vi "Window-Position control window.vi"() -> ()   [LabVIEW 2020]
uses:
  <userlib>/My Palettes.lib/Custom Controls/Directional Arrow Buttons/Arrow button-East.ctl
  <userlib>/My Palettes.lib/Custom Controls/Directional Arrow Buttons/Arrow button-West.ctl
  <userlib>/My Palettes.lib/Custom Controls/Directional Arrow Buttons/Arrow button-North.ctl
  <userlib>/My Palettes.lib/Custom Controls/Directional Arrow Buttons/Arrow button-South.ctl
  <userlib>/My Palettes.lib/Custom Controls/Directional Arrow Buttons/Arrow button-North west.ctl
  <userlib>/My Palettes.lib/Custom Controls/Directional Arrow Buttons/Arrow button-North east.ctl
  <userlib>/My Palettes.lib/Custom Controls/Directional Arrow Buttons/Arrow button-South west.ctl
  <userlib>/My Palettes.lib/Custom Controls/Directional Arrow Buttons/Arrow button-South east.ctl
  User Interface/Windows/Position control window/Typedefs/Pos Ctrl States.ctl
  User Interface/Windows/Position control window/Typedefs/Pos Ctrl queue data cluster.ctl
  User Interface/Windows/Position control window/Typedefs/Pos Ctrl window refs cluster.ctl
  Typedefs/Movement mode.ctl
  Peripherals Control/XYZ Stage/Typedefs/XYZ stage states.ctl
  Typedefs/Axis of movement.ctl
  User Interface/Windows/Position control window/Globals/Pos ctrl window globals.vi
  Global Variables/General Globals.vi
  Peripherals Control/XYZ Stage/Globals/gl_XYZStage globals.vi
  Typedefs/Save-Load enum.ctl
  Peripherals Control/XYZ Stage/Typedefs/XYZ channel ring.ctl
  Peripherals Control/XYZ Stage/Typedefs/XYZ stage data.ctl
panel:
  in  "Speed setting\navailable":bool
  in  "Motor E-Stop":bool
  out "# elements in queue":i32
  out "x+1":dbl
  in  "Y Coordinate ctrl":sgl min=-20000 max=20000 step=0.1 format="Y:%#_g um"
  out "Close":bool
  in  "Z step (um)":sgl=1.0 min=0.1 max=1000 step=0.1 format="%#_6f"
  in  "Z Coordinate ctrl":sgl min=-20000 max=20000 step=0.1 format="Z:%#.1f um"
  in  "Z move down":T1
  in  "Z move up":T2
  out "Z-axis section":string
  in  "Step = size of image":bool
  in  "XY step (um)":sgl=1.0 min=0.1 max=10000 step=0.1
  out "State":T3
  out "Last button name":string
  out "Event loop":i32
  out "Elapsed Time (s)":dbl format="%#.1g"
  in  "Speed setting ctrl":i32=1000 min=1000 max=50000 step=1 format="Speed\n%#_6g\num/sec"
  in  "Speed down":bool
  in  "Speed up":bool
  in  "X Coordinate ctrl":sgl min=-20000 max=20000 step=0.1 format="X:%#_g um"
  in  "Down-right":T4
  in  "Down-left":T5
  in  "Up-right":T6
  in  "Up-left":T7
  in  "Down":T1
  in  "Up":T2
  in  "Left":T8
  in  "Right":T9
  # "Speed"
  # "X-Y Movement"
  # "Z Movement"
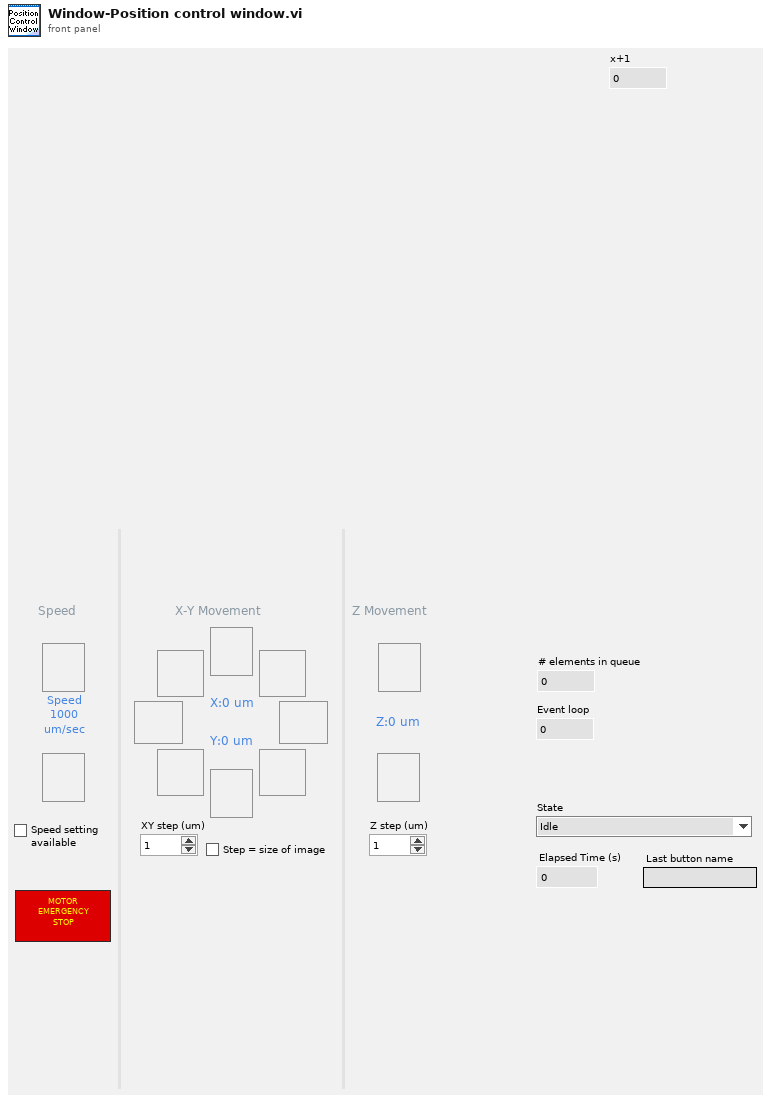
[diagram p1: front panel]
types:
  T1 = typedef "Arrow button-South.ctl" = bool
  T2 = typedef "Arrow button-North.ctl" = bool
  T3 = typedef "Pos Ctrl States.ctl" = enum16{"Idle", "Count-down", "Request single step (ack.)", "Request single step (no ack.)", "Request continuous movement", "Request movement stop"}
  T4 = typedef "Arrow button-South east.ctl" = bool
  T5 = typedef "Arrow button-South west.ctl" = bool
  T6 = typedef "Arrow button-North east.ctl" = bool
  T7 = typedef "Arrow button-North west.ctl" = bool
  T8 = typedef "Arrow button-West.ctl" = bool
  T9 = typedef "Arrow button-East.ctl" = bool
  T10 = typedef "Pos Ctrl window refs cluster.ctl" = cluster{"menu reference":refnum<k9>, "X Coordinate ctrl":refnum<vi>, "Y Coordinate ctrl":refnum<vi>, "Z Coordinate ctrl":refnum<vi>, "Speed setting ctrl":refnum<vi>, "Up":refnum<vi>, "Down":refnum<vi>, "Left":refnum<vi>, "Right":refnum<vi>, "Z move up":refnum<vi>, "Z move down":refnum<vi>, "Down-left":refnum<vi>, "Down-right":refnum<vi>, "Up-left":refnum<vi>, "Up-right":refnum<vi>, "Step = size of image":refnum<vi>, "XY step (um)":refnum<vi>, "Z step (um)":refnum<vi>, "Speed setting\navailable":refnum<vi>}
  T11 = typedef "Pos Ctrl queue data cluster.ctl" = cluster{"State":T3, "variant":variant}
  T12 = enum32{"Invalid", "Standard", "Closed", "Hidden", "Minimized", "Maximized"}
  T13 = typedef "XYZ stage states.ctl" = enum16{"Dequeue", "Initialize", "Read Position", "Read Speed Setting", "Move", "Set Max Speed", "Reset Axis", "Stop all movement"}
  T14 = typedef "Axis of movement.ctl" = enum16{"None", "X-axis", "Y-Axis", "-45 deg Axis", "+45 deg Axis", "Z-Axis"}
  T15 = enum8{"Enabled", "Disabled", "Disabled and Grayed Out"}
  T16 = typedef "XYZ stage data.ctl" = cluster{"Command":T13, "Channel":T17, "X":sgl, "Y":sgl, "Z":sgl, "Speed":i32, "Zero":bool, "Use acknowledgement?":bool}
  T17 = typedef "XYZ channel ring.ctl" = string
  T18 = typedef "Save-Load enum.ctl" = enum16{"Save to file", "Load from file", "Compare from file", "Save Backup"}
  T19 = typedef "Movement mode.ctl" = enum16{"Move the frame", "Move the feature"}
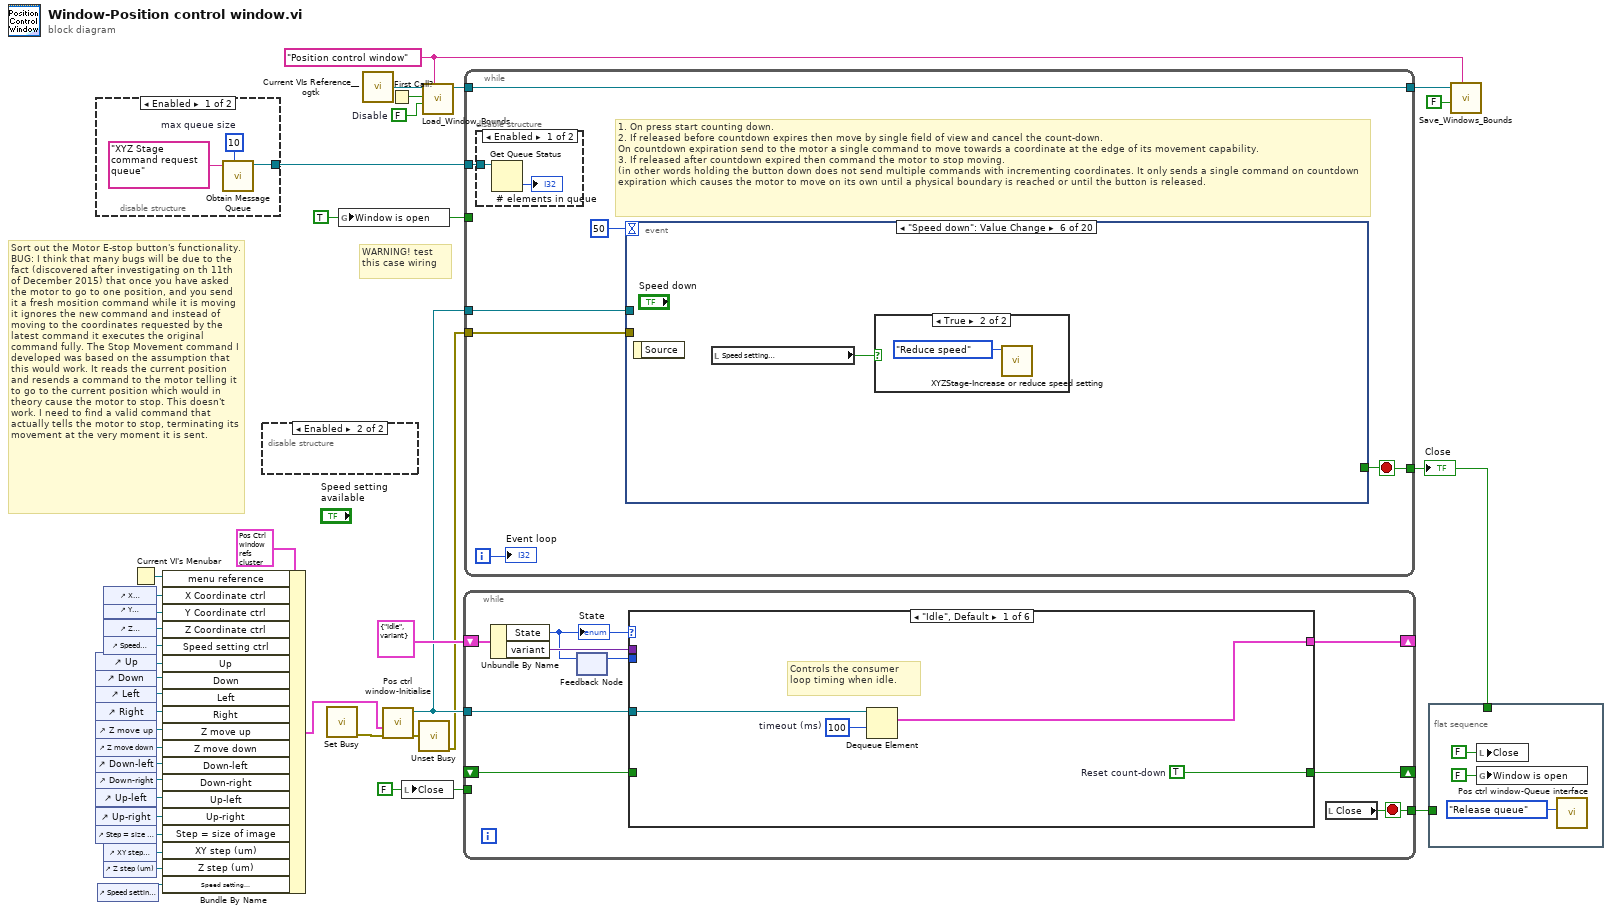
[diagram p0: block diagram]
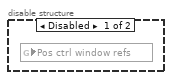
[diagram p3: hidden frame]
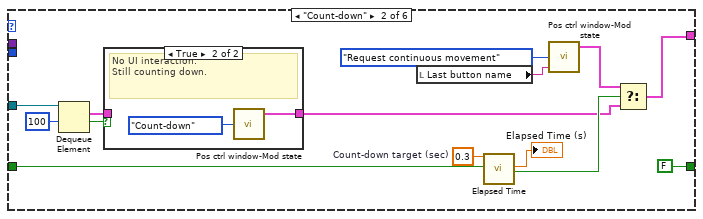
[diagram p4: hidden frame]
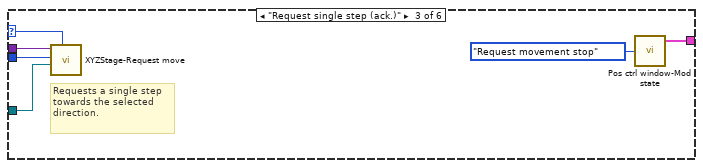
[diagram p6: hidden frame]
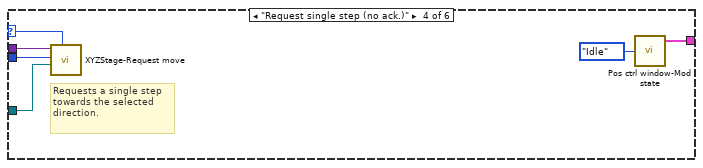
[diagram p7: hidden frame]
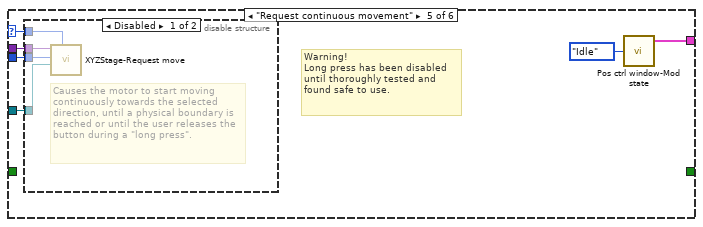
[diagram p8: hidden frame]
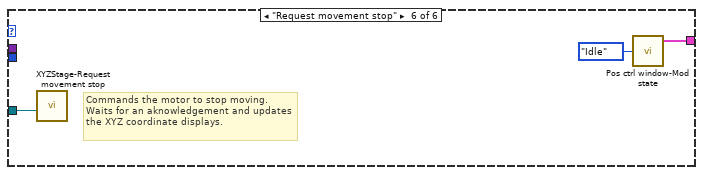
[diagram p10: hidden frame]
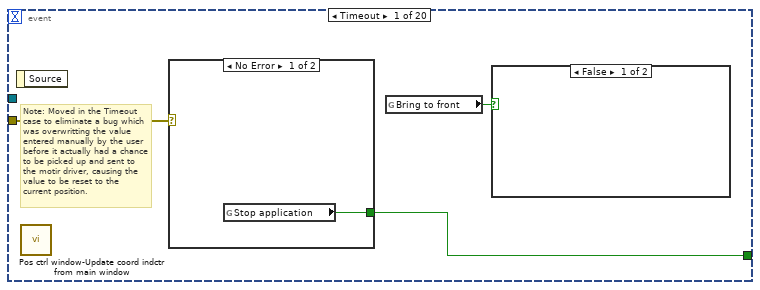
[diagram p12: hidden frame]
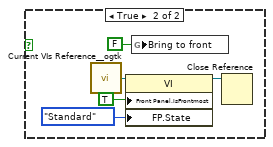
[diagram p13: hidden frame]
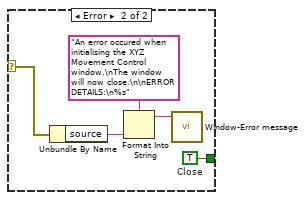
[diagram p14: hidden frame]
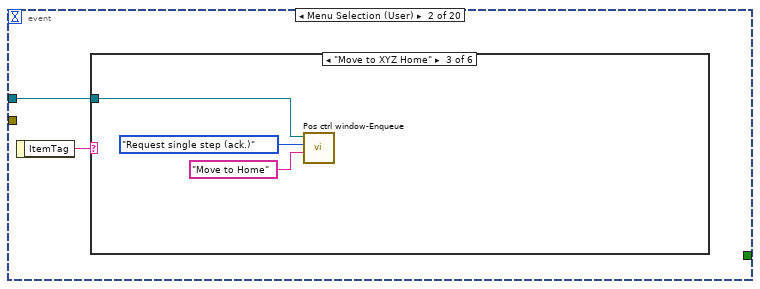
[diagram p15: hidden frame]
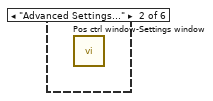
[diagram p17: hidden frame]
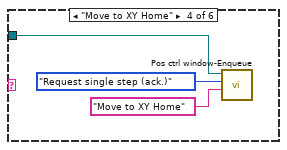
[diagram p18: hidden frame]
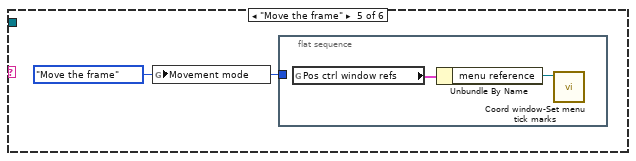
[diagram p19: hidden frame]
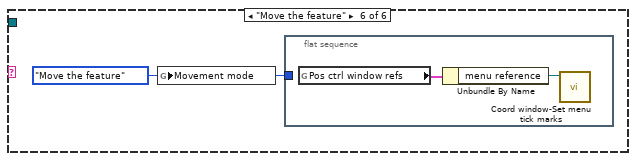
[diagram p20: hidden frame]
diagram:
  w11 = FALSE  # Disable
  w9 = "Position control window" ("Window Name (i.e. Key)")
  w15 = TRUE ("Bring to front")
  w26 = FALSE ("Close")
  # "Sort out the Motor E-stop button's functionality.\nBUG: I think that many bugs will be due to the fact (discovered after investigating on th 11th of December 2015) that once you have asked the motor to go to one position, and you send it a fresh mosition command while it is moving it ignores the new command and instead of moving to the coordinates requested by the latest command it executes the original command fully. The Stop Movement command I developed was based on the assumption that this would work. It reads the current position and resends a command to the motor telling it to go to the current position which would in theory cause the motor to stop. This doesn't work. I need to find a valid command that actually tells the motor to stop, terminating its movement at the very moment it is sent."
  # "WARNING! test this case wiring"
  n1 = control-ref of="Up"() -> (w36:refnum<vi>)
  n2 = control-ref of="Down"() -> (w35:refnum<vi>)
  n3 = control-ref of="Left"() -> (w34:refnum<vi>)
  n4 = control-ref of="Right"() -> (w33:refnum<vi>)
  n5 = control-ref of="Z move up"() -> (w32:refnum<vi>)
  n6 = control-ref of="Z move down"() -> (w31:refnum<vi>)
  n7 = control-ref of="Down-left"() -> (w30:refnum<vi>)
  n8 = control-ref of="Down-right"() -> (w29:refnum<vi>)
  n9 = control-ref of="Up-left"() -> (w28:refnum<vi>)
  n10 = control-ref of="Up-right"() -> (w27:refnum<vi>)
  n11 = control-ref of="Step = size of image"() -> (w24:refnum<vi>)
  n12 = disable-structure shown="Enabled" {
    disable-tunnel: [w39 _] -> w7
    frame Enabled {
      w41 = 10  # max queue size
      n13 = call "Obtain Message Queue.vi"("max queue size (-1, unlimited)"=w41, "Queue name"="XYZ Stage command request queue") -> ("Message Queue"=w39:refnum<queue>)  [unwired: 8 in, 1 out]
    }
    frame Disabled {
    }
  }
  n14 = control-ref of="Speed setting\navailable"() -> (w1:refnum<vi>)
  n15 = control-ref of="X Coordinate ctrl"() -> (w19:refnum<vi>)
  n16 = control-ref of="Y Coordinate ctrl"() -> (w18:refnum<vi>)
  n17 = control-ref of="Z Coordinate ctrl"() -> (w17:refnum<vi>)
  n18 = control-ref of="Speed setting ctrl"() -> (w16:refnum<vi>)
  n19 = control-ref of="XY step (um)"() -> (w23:refnum<vi>)
  n20 = control-ref of="Z step (um)"() -> (w22:refnum<vi>)
  n21 = Current VI's Menubar() -> (w6:refnum<k9>)
  n22 = Bundle By Name(cluster=T10 {"menu reference"=refnum, "X Coordinate ctrl"=refnum, "Y Coordinate ctrl"=refnum, "Z Coordinate ctrl"=refnum, "Speed setting ctrl"=refnum, "Up"=refnum, "Down"=refnum, "Left"=refnum, "Right"=refnum, "Z move up"=refnum, "Z move down"=refnum, "Down-left"=refnum, "Down-right"=refnum, "Up-left"=refnum, "Up-right"=refnum, "Step = size of image"=refnum, "XY step (um)"=refnum, "Z step (um)"=refnum, "Speed setting\navailable"=refnum} ("Pos ctrl window refs"), "menu reference"=w6, "X Coordinate ctrl"=w19, "Y Coordinate ctrl"=w18, "Z Coordinate ctrl"=w17, "Speed setting ctrl"=w16, "Up"=w36, "Down"=w35, "Left"=w34, "Right"=w33, "Z move up"=w32, "Z move down"=w31, "Down-left"=w30, "Down-right"=w29, "Up-left"=w28, "Up-right"=w27, "Step = size of image"=w24, "XY step (um)"=w23, "Z step (um)"=w22, "Speed setting\navailable"=w1) -> (w20:T10)
  n23 = disable-structure shown="Enabled" {
    frame Disabled {
      n24 = global read "Pos ctrl window globals.vi" "Pos ctrl window refs"() -> ()  [unwired: 1 in]
    }
    frame Enabled {
    }
  }
  n25 = call <vilib>:"Set Busy.vi"() -> ("error out"=w4:errorcluster)  [unwired: 10 in, 1 out]
  n26 = global write "Pos ctrl window globals.vi" "Window is open"(w15) -> ()
  n27 = call <userlib>:"Current VIs Reference__ogtk.vi"() -> ("Current VI's reference"=w14:refnum<vi>)  [unwired: 5 in]
  n28 = call "Pos ctrl window-Initialise.vi"("error in (no error)"=w4, "Pos ctrl window refs"=w20) -> ("error out"=w3:errorcluster, "XYZ movement ctrl window queue ref"=w21:refnum<queue>)  [unwired: 8 in]
  n29 = First Call?() -> (First Call?: T/F=w12:bool)
  n30 = local write "Close"(w26) -> ()
  n31 = call <vilib>:"Unset Busy.vi"("error in (no error)"=w3) -> ("error out"=w2:errorcluster)  [unwired: 10 in]
  n32 = call "Load_Window_Bounds.vi"("Window Name (i.e. Key)"=w9, "Disable"=w11, "First Call"=w12, "Window VI's Ref"=w14) -> ("reference out"=w13:refnum<vi>)  [unwired: 4 in, 3 out]
  n33 = while {
    tunnel: w21 -> [w50]
    shift-right: [w49] -> _
    shift-left: T11 {"State"=enum."Idle", "variant"=variant} ("Pos Ctrl queue data cluster") -> [w46]
    shift-right: [w48] -> _
    shift-left: _ -> [w47]
    tunnel: w26 -> [_]
    tunnel: [w42] -> w25
    stop <- w42 stop-if-true
    n34 = Unbundle By Name(w46) -> ("State"=w44:T3, "variant"=w45:variant)
    "State" <- w44
    n35 = feedback-in #1(w44) -> ()
    n36 = feedback #1() -> (w43:T3)  [unwired: 1 in]
    n37 = case shown="\"Idle\", Default" w44 {
      selector: w44 -> [_ _ w72 w78 w84 _]
      tunnel: w50 -> [w53 w67 w74 w80 w87 w94]
      tunnel: [w51 w56 w76 w82 w88 w95] -> w49
      tunnel: [w52 FALSE _ _ _ _] -> w48
      tunnel: w47 -> [_ w64 _ _ _ _]
      tunnel: w45 -> [_ _ w75 w81 w86 _]
      tunnel: w43 -> [_ _ w73 w79 w85 _]
      frame "Idle", Default {
        w52 = TRUE  # Reset count-down
        w54 = 100  # timeout (ms)
        # "Controls the consumer loop timing when idle."
        n38 = Dequeue Element(queue=w53, timeout in ms (-1)=w54) -> (element=w51:T11)  [unwired: 1 in, 3 out]
      }
      frame "Count-down" {
        w65 = 0.3  # Count-down target (sec)
        n39 = Dequeue Element(queue=w67, timeout in ms (-1)=100) -> (element=w62:T11, timed out?=w63:bool)  [unwired: 1 in, 2 out]
        n40 = case shown="True" w63 {
          tunnel: [w69 w70] -> w57
          tunnel: w62 -> [w69 _]
          frame False {
            # "Queue element received.\nUI interaction detected."
          }
          frame True {
            # "No UI interaction.\nStill counting down."
            n41 = call "Pos ctrl window-Mod state.vi"("States"=Pos_Ctrl_States."Count-down") -> ("Modified queue element"=w70:T11)  [unwired: 4 in]
          }
        }
        n42 = local read "Last button name"() -> (w55:string)
        n43 = call "Elapsed Time"("Time Target (s)"=w65, "Reset"=w64) -> ("Elapsed Time (s)"=→"Elapsed Time (s)":dbl, "Time has Elapsed"=w58:bool)  [unwired: 10 in, 6 out]
        n44 = call "Pos ctrl window-Mod state.vi"("variant"=w55, "States"=Pos_Ctrl_States."Request continuous movement") -> ("Modified queue element"=w60:T11)  [unwired: 3 in]
        n45 = Select(t=w60, s=w58, f=w57) -> (s? t:f=w56:T11)
      }
      frame "Request single step (ack.)" {
        # "Requests a single step towards the selected direction."
        n46 = call "XYZStage-Request move.vi"("Current State"=w72, "Pos ctrl window queue"=w74, "Previous State"=w73, "variant"=w75) -> ()  [unwired: 8 in]
        n47 = call "Pos ctrl window-Mod state.vi"("States"=Pos_Ctrl_States."Request movement stop") -> ("Modified queue element"=w76:T11)  [unwired: 4 in]
      }
      frame "Request single step (no ack.)" {
        # "Requests a single step towards the selected direction."
        n48 = call "XYZStage-Request move.vi"("Current State"=w78, "Pos ctrl window queue"=w80, "Previous State"=w79, "variant"=w81) -> ()  [unwired: 8 in]
        n49 = call "Pos ctrl window-Mod state.vi"("States"=Pos_Ctrl_States."Idle") -> ("Modified queue element"=w82:T11)  [unwired: 4 in]
      }
      frame "Request continuous movement" {
        # "Warning!\nLong press has been disabled until thoroughly tested and found safe to use."
        n50 = disable-structure shown="Disabled" {
          disable-tunnel: w87 -> [w93 _]
          disable-tunnel: w86 -> [w92 _]
          disable-tunnel: w85 -> [w91 _]
          disable-tunnel: w84 -> [w90 _]
          frame Disabled {
            # "Causes the motor to start moving continuously towards the selected direction, until a physical boundary is reached or until the user releases the button during a \"long press\"."
            n51 = call "XYZStage-Request move.vi"("Current State"=w90, "Pos ctrl window queue"=w93, "Previous State"=w91, "variant"=w92) -> ()  [unwired: 8 in]
          }
          frame Enabled {
          }
        }
        n52 = call "Pos ctrl window-Mod state.vi"("States"=Pos_Ctrl_States."Idle") -> ("Modified queue element"=w88:T11)  [unwired: 4 in]
      }
      frame "Request movement stop" {
        # "Commands the motor to stop moving.\nWaits for an aknowledgement and updates the XYZ coordinate displays."
        n53 = call "XYZStage-Request movement stop.vi"("Pos ctrl window queue"=w94) -> ()  [unwired: 11 in]
        n54 = call "Pos ctrl window-Mod state.vi"("States"=Pos_Ctrl_States."Idle") -> ("Modified queue element"=w95:T11)  [unwired: 4 in]
      }
    }
    n55 = local read "Close"() -> (w42:bool)
  }
  n56 = while {
    tunnel: w21 -> [w102]
    tunnel: [w100] -> w5
    tunnel: w2 -> [w99]
    tunnel: w15 -> [_]
    tunnel: w13 -> [w98]
    tunnel: [w98] -> w10
    tunnel: w7 -> [w97]
    i -> [w101]
    stop <- w100 stop-if-true
    # "1. On press start counting down.\n2. If released before countdown expires then move by single field of view and cancel the count-down.\nOn countdown expiration send to the motor a single command to move towards a coordinate at the edge of its movement capability.\n3. If released after countdown expired then command the motor to stop moving.\n(in other words holding the button down does not send multiple commands with incrementing coordinates. It only sends a single command on countdown expiration which causes the motor to move on its own until a physical boundary is reached or until the button is released."
    n57 = disable-structure shown="Enabled" {
      disable-tunnel: w97 -> [w105 _]
      frame Enabled {
        n58 = Get Queue Status(queue=w105) -> (# elements in queue=→"# elements in queue":i32)  [unwired: 2 in, 7 out]
      }
      frame Disabled {
      }
    }
    n59 = event shown="[5] \"Speed down\": Value Change" {
      selector: _ -> [_ _ _ _ _ _ _ _ _ _ _ _ _ _ _ _ _ _ _ _]
      dyn-events: _ -> [_ _ _ _ _ _ _ _ _ _ _ _ _ _ _ _ _ _ _ _]
      timeout: 50 -> [_ _ _ _ _ _ _ _ _ _ _ _ _ _ _ _ _ _ _ _]
      tunnel: w102 -> [_ w120 w137 _ _ _ w177 w180 w188 _ _ _ _ _ _ _ _ _ w204 _]
      tunnel: [w107 _ _ _ _ _ _ _ _ _ _ _ _ _ _ _ _ _ _ TRUE] -> w100
      tunnel: w99 -> [w108 _ _ _ _ _ _ _ _ _ _ _ _ _ _ _ _ _ _ _]
      event Timeout {
        # "Note: Moved in the Timeout case to eliminate a bug which was overwritting the value entered manually by the user before it actually had a chance to be picked up and sent to the motir driver, causing the value to be reset to the current position."
        n60 = event-data() -> ()  [unwired: 1 in, 1 out]
        n61 = call "Pos ctrl window-Update coord indctr from main window.vi"() -> ()  [unwired: 12 in]
        n62 = case shown="No Error" w108 {
          selector: w108 -> [_ w116]
          tunnel: [w114 w119] -> w107
          frame No Error {
            n63 = global read "General Globals.vi" "Stop application"() -> (w114:bool)
          }
          frame Error {
            w119 = TRUE  # Close
            n64 = Unbundle By Name(w116) -> ("source"=w115:string)
            n65 = Format Into String(format string="An error occured when initialising the XYZ Movement Control window.\nThe window will now close.\n\nERROR DETAILS:\n%s" ("Error Source"), w115) -> (resulting string=w118:string)  [unwired: 2 in, 1 out]
            n66 = call "Window-Error message.vi"("Message"=w118) -> ()  [unwired: 10 in, 1 out]
          }
        }
        n67 = global read "Pos ctrl window globals.vi" "Bring to front"() -> (w106:bool)
        n68 = case shown="False" w106 {
          frame False {
          }
          frame True {
            n69 = call <userlib>:"Current VIs Reference__ogtk.vi"() -> ("Current VI's reference"=w112:refnum<vi>)  [unwired: 5 in]
            n70 = property class="VI"(reference=w112, "Front Panel.IsFrontmost"=TRUE ("Front Panel Window:Is Frontmost"), "FP.State"=T12."Standard" ("Front Panel Window:State")) -> (reference out=w111:refnum<vi>)  [unwired: 1 in, 1 out]
            n71 = global write "Pos ctrl window globals.vi" "Bring to front"(FALSE ("Bring to front")) -> ()
            n72 = Close Reference(reference=w111) -> ()  [unwired: 1 in, 1 out]
          }
        }
      }
      event Menu Selection (User) {
        n73 = event-data() -> ("ItemTag"=w121:string)  [unwired: 1 in]
        n74 = case shown="\"Move to XYZ Home\"" w121 {
          tunnel: w120 -> [_ _ w122 w125 _ _]
          frame Default {
          }
          frame "Advanced Settings..." {
            n75 = call "Pos ctrl window-Settings window.vi"() -> ()  [unwired: 11 in, 1 out]
          }
          frame "Move to XYZ Home" {
            n76 = call "Pos ctrl window-Enqueue.vi"("variant"="Move to Home" ("Last button name"), "States"=Pos_Ctrl_States."Request single step (ack.)", "Pos ctrl window queue"=w122) -> ()  [unwired: 8 in, 1 out]
          }
          frame "Move to XY Home" {
            n77 = call "Pos ctrl window-Enqueue.vi"("variant"="Move to XY Home" ("Last button name"), "States"=Pos_Ctrl_States."Request single step (ack.)", "Pos ctrl window queue"=w125) -> ()  [unwired: 8 in, 1 out]
          }
          frame "Move the frame" {
            w128 = Movement_mode."Move the frame" ("Movement mode")
            n78 = global write "Pos ctrl window globals.vi" "Movement mode"(w128) -> ()
            n79 = flat-sequence {
              tunnel: w128 -> [_]
              frame #0 {
                n80 = global read "Pos ctrl window globals.vi" "Pos ctrl window refs"() -> (w129:T10)
                n81 = Unbundle By Name(w129) -> ("menu reference"=w130:refnum<k9>)
                n82 = call "Coord window-Set menu tick marks.vi"("Menu in"=w130) -> ()  [unwired: 9 in, 2 out]
              }
            }
          }
          frame "Move the feature" {
            w131 = Movement_mode."Move the feature" ("Movement mode")
            n83 = global write "Pos ctrl window globals.vi" "Movement mode"(w131) -> ()
            n84 = flat-sequence {
              tunnel: w131 -> [_]
              frame #0 {
                n85 = global read "Pos ctrl window globals.vi" "Pos ctrl window refs"() -> (w132:T10)
                n86 = Unbundle By Name(w132) -> ("menu reference"=w133:refnum<k9>)
                n87 = call "Coord window-Set menu tick marks.vi"("Menu in"=w133) -> ()  [unwired: 9 in, 2 out]
              }
            }
          }
        }
      }
      event Mouse Wheel {
        # "Controls the stage when scrolling the mouse wheel over the Up or Down arrow key."
        n88 = event-data() -> ("Delta"=w136:i32)  [unwired: 1 in]
        n89 = global read "Pos ctrl window globals.vi" "Axis of movement"() -> (w134:T14)
        n90 = Greater Than 0?(x=w136) -> (x > 0?=w135:bool)
        n91 = case shown="Default" w134 {
          selector: w134 -> [_ w138]
          tunnel: w137 -> [_ w144]
          tunnel: w135 -> [_ w142]
          frame "None" {
          }
          frame Default {
            n92 = case shown="\"Z-Axis\"" w138 {
              tunnel: [w146 w150 w154 w159 w163] -> w143
              tunnel: w142 -> [w147 w151 w155 w158 w162]
              frame "X-axis", Default {
                n93 = case shown="True" w147 {
                  tunnel: ["Left" "Right"] -> w146
                  frame False {
                    # "Reducing X"
                  }
                  frame True {
                    # "Increasing X"
                  }
                }
              }
              frame "-45 deg Axis" {
                n94 = case shown="True" w151 {
                  tunnel: ["Down-right" "Up-left"] -> w150
                  frame False {
                  }
                  frame True {
                  }
                }
              }
              frame "+45 deg Axis" {
                n95 = case shown="True" w155 {
                  tunnel: ["Down-left" "Up-right"] -> w154
                  frame False {
                  }
                  frame True {
                  }
                }
              }
              frame "Y-Axis" {
                n96 = case shown="True" w158 {
                  tunnel: ["Down" "Up"] -> w159
                  frame False {
                    # "Reducing Y"
                  }
                  frame True {
                    # "Increasing Y"
                  }
                }
              }
              frame "Z-Axis" {
                n97 = case shown="False" w162 {
                  tunnel: ["Z move down" "Z move up"] -> w163
                  frame False {
                    # "Reducing Z"
                  }
                  frame True {
                    # "Increasing Z"
                  }
                }
              }
            }
            n98 = local write "Last button name"(w143) -> ()
            n99 = feedback #2(0.0) -> (w141:dbl)
            n100 = Increment(x=w141) -> (x+1=w140:dbl)
            "x+1" <- w140
            n101 = feedback-in #2(w140) -> ()
            n102 = call "Pos ctrl window-Enqueue.vi"("variant"=w143, "States"=Pos_Ctrl_States."Request single step (no ack.)", "Pos ctrl window queue"=w144) -> ()  [unwired: 8 in, 1 out]
          }
        }
      }
      event "Speed setting ctrl": Value Change {
        n103 = event-data() -> ("NewVal"=w167:i32)  [unwired: 1 in]
        n104 = local read "Speed setting\navailable"() -> (w166:bool)
        n105 = case shown="True" w166 {
          tunnel: w167 -> [_ w168]
          frame False {
          }
          frame True {
            n106 = call "XYZStage-Request speed setting command.vi"("Speed to set"=w168, "Which speed setting command?"=XYZ_stage_states."Set Max Speed" ("Command")) -> ()  [unwired: 9 in, 1 out]
          }
        }
      }
      event "Speed up": Value Change {
        n107 = event-data() -> ()  [unwired: 1 in, 1 out]
        n108 = local read "Speed setting\navailable"() -> (w170:bool)
        n109 = case shown="True" w170 {
          frame False {
          }
          frame True {
            n110 = call "XYZStage-Increase or reduce speed setting.vi"("Function"=enum16{"Increase speed", "Reduce speed"}."Increase speed") -> ()  [unwired: 11 in]
          }
        }
      }
      event "Speed down": Value Change {
        n111 = event-data() -> ()  [unwired: 1 in, 1 out]
        n112 = local read "Speed setting\navailable"() -> (w172:bool)
        n113 = case shown="True" w172 {
          frame False {
          }
          frame True {
            n114 = call "XYZStage-Increase or reduce speed setting.vi"("Function"=enum16{"Increase speed", "Reduce speed"}."Reduce speed") -> ()  [unwired: 11 in]
          }
        }
      }
      event Mouse Down {
        # "WARNING!\nDO NOT CHANGE THE CONTROL NAMES.\nIF YOU DO MAKE SURE YOU ALSO UPDATE\nTHE \"XYZStage-Request single step.vi\""
        # "Handles all directional buttons including the Z-axis buttons."
        n115 = event-data() -> ("CtlRef"=w175:refnum<vi>)  [unwired: 1 in]
        n116 = property class="Bool (strict)"(reference=w175) -> ("Label.Text"=w174:string)  [unwired: 1 in, 2 out]
        "Last button name" <- w174
        n117 = call "Pos ctrl window-Enqueue.vi"("variant"=w174, "States"=Pos_Ctrl_States."Count-down", "Pos ctrl window queue"=w177) -> ()  [unwired: 8 in, 1 out]
      }
      event "Z Coordinate ctrl", "X Coordinate ctrl", "Y Coordinate ctrl": Value Change {
        n118 = event-data() -> ("CtlRef"=w179:refnum<vi>)  [unwired: 1 in]
        n119 = property class="DigNum (strict)"(reference=w179) -> ("Label.Text"=w178:string)  [unwired: 1 in, 2 out]
        n120 = local write "Last button name"(w178) -> ()
        n121 = call "Pos ctrl window-Enqueue.vi"("variant"=w178, "States"=Pos_Ctrl_States."Request single step (ack.)", "Pos ctrl window queue"=w180) -> ()  [unwired: 8 in, 1 out]
      }
      event Mouse Up {
        # "Also bundles the name of the control.\nThis is then used to determine the direction.\nHandles all the directional buttons."
        # "Handles all directional buttons including the Z-axis buttons."
        n122 = event-data() -> ("CtlRef"=w187:refnum<vi>)  [unwired: 1 in]
        n123 = local read "State"() -> (w185:T3)
        n124 = Equal?(x=Pos_Ctrl_States."Count-down", y=w185) -> (x = y?=w183:bool)
        n125 = case shown="True" w183 {
          tunnel: [Pos_Ctrl_States."Request movement stop" ("States") Pos_Ctrl_States."Request single step (ack.)" ("States")] -> w182
          frame False {
            # "Long-press count down has completed"
          }
          frame True {
            # "Still in count-down for long-press"
          }
        }
        n126 = property class="Bool (strict)"(reference=w187) -> ("Label.Text"=w186:string)  [unwired: 1 in, 2 out]
        n127 = local write "Last button name"(w186) -> ()
        n128 = call "Pos ctrl window-Enqueue.vi"("variant"=w186, "States"=w182, "Pos ctrl window queue"=w188) -> ()  [unwired: 8 in, 1 out]
      }
      event "Y Coordinate ctrl": Mouse Enter {
        n129 = event-data() -> ()  [unwired: 1 in, 1 out]
        n130 = global write "Pos ctrl window globals.vi" "Axis of movement"(Axis_of_movement."Y-Axis" ("Axis of movement")) -> ()
      }
      event "X Coordinate ctrl": Mouse Enter {
        n131 = event-data() -> ()  [unwired: 1 in, 1 out]
        n132 = global write "Pos ctrl window globals.vi" "Axis of movement"(Axis_of_movement."X-axis" ("Axis of movement")) -> ()
      }
      event Mouse Enter {
        n133 = event-data() -> ()  [unwired: 1 in, 1 out]
        n134 = global write "Pos ctrl window globals.vi" "Axis of movement"(Axis_of_movement."-45 deg Axis" ("Axis of movement")) -> ()
      }
      event Mouse Enter {
        n135 = event-data() -> ()  [unwired: 1 in, 1 out]
        n136 = global write "Pos ctrl window globals.vi" "Axis of movement"(Axis_of_movement."+45 deg Axis" ("Axis of movement")) -> ()
      }
      event "Z-axis section": Mouse Enter {
        # "This indicator is hidden and causes the Z-slider to come in focus on a \"mouse enter\" event."
        n137 = event-data() -> ()  [unwired: 1 in, 1 out]
        n138 = global write "Pos ctrl window globals.vi" "Axis of movement"(Axis_of_movement."Z-Axis" ("Axis of movement")) -> ()
      }
      event "Speed up", "Speed down", "Z-axis section", "X Coordinate ctrl", "Y Coordinate ctrl": Mouse Leave {
        n139 = event-data() -> ()  [unwired: 1 in, 1 out]
        n140 = global write "Pos ctrl window globals.vi" "Axis of movement"(Axis_of_movement."None" ("Axis of movement")) -> ()
      }
      event "XY step (um)": Value Change {
        n141 = event-data() -> ()  [unwired: 1 in, 1 out]
        n142 = global write "Pos ctrl window globals.vi" "XY step (um)"("XY step (um)") -> ()
      }
      event "Z step (um)": Value Change {
        n143 = event-data() -> ()  [unwired: 1 in, 1 out]
        n144 = global write "Pos ctrl window globals.vi" "Z step (um)"("Z step (um)") -> ()
      }
      event "Step = size of image": Value Change {
        n145 = event-data() -> ()  [unwired: 1 in, 1 out]
        n146 = global write "Pos ctrl window globals.vi" "Step = size of image"("Step = size of image") -> ()
        n147 = Select(t=T15."Disabled and Grayed Out" ("Disabled"), s="Step = size of image", f=T15."Enabled" ("Disabled")) -> (s? t:f=w201:T15)
        n148 = property on="XY step (um)" class="DigNum (strict)"("DisabledEnum"=w201) -> ()  [unwired: 2 in, 2 out]
      }
      event "Motor E-Stop": Value Change {
        n149 = event-data() -> ()  [unwired: 1 in, 1 out]
        n150 = Flush Queue(queue=w204) -> (error out=w203:errorcluster)  [unwired: 1 in, 2 out]
        n151 = flat-sequence {
          tunnel: w203 -> [_]
          frame #0 {
            n152 = disable-structure shown="Enabled" {
              frame Disabled {
                n153 = Bundle By Name(cluster=T16 {"Command"=enum."Initialize", "Channel"="Z", "X"=0.0, "Y"=0.0, "Z"=0.0, "Speed"=0, "Zero"=FALSE, "Use acknowledgement?"=FALSE} ("XYZ Stage data to queue"), "Use acknowledgement?"=FALSE) -> (w208:T16)
                n154 = call "XYZ Stage-Command request module.vi"("Command"=XYZ_stage_states."Stop all movement", "XYZ Stage data to queue"=w208) -> ()  [unwired: 5 in, 5 out]
              }
              frame Enabled {
                n155 = global write "gl_XYZStage globals.vi" "Motor E-stop"(TRUE ("Motor E-stop")) -> ()
              }
            }
          }
        }
      }
      event Panel Close {
        # "The XYZ window setup is now saved as part of the user-profile save functionality and no longer auto-saved when the window is closed."
        n156 = event-data() -> ()  [unwired: 1 in, 1 out]
        n157 = disable-structure shown="Disabled" {
          frame Disabled {
            n158 = call "Read-Write XYZ movement setup.vi"("Function"=Save-Load_enum."Save to file") -> ()  [unwired: 10 in, 1 out]
          }
          frame Enabled {
          }
        }
      }
    }
    "Event loop" <- w101
  }
  "Close" <- w5
  n159 = flat-sequence {
    tunnel: w25 -> [_]
    tunnel: w5 -> [_]
    frame #0 {
      n160 = local write "Close"(FALSE ("Close")) -> ()
      n161 = global write "Pos ctrl window globals.vi" "Window is open"(FALSE ("Bring to front")) -> ()
      n162 = call "Pos ctrl window-Queue interface.vi"("Function"=enum16{"None", "Release queue"}."Release queue") -> ()  [unwired: 9 in, 2 out]
    }
  }
  n163 = call "Save_Windows_Bounds.vi"("Window Name (i.e. Key)"=w9, "Front Panel Window:Open"=FALSE, "Window VI's Ref"=w10) -> ()  [unwired: 8 in, 1 out]
